vi "RDV-linkPlotVisibility.vi"(8 "error in (no error)":errorcluster, 11 "RDV-Reflection_Data_viewer in":refnum<class "RDV-Reflection_Data_viewer.lvclass">) -> (0 "error out":errorcluster, 3 "RDV-Reflection_Data_viewer out":refnum<class "RDV-Reflection_Data_viewer.lvclass">)   [LabVIEW 2020, in "RDV-Reflection_Data_viewer.lvclass"]
doc: "Links the plot visibility between the viewer's graphs."
uses:
  RDV-Reflection_Data_viewer.lvclass
  RDV-Reflection_Data_viewer.lvclass/RDV-Reflection_Data_viewer.ctl
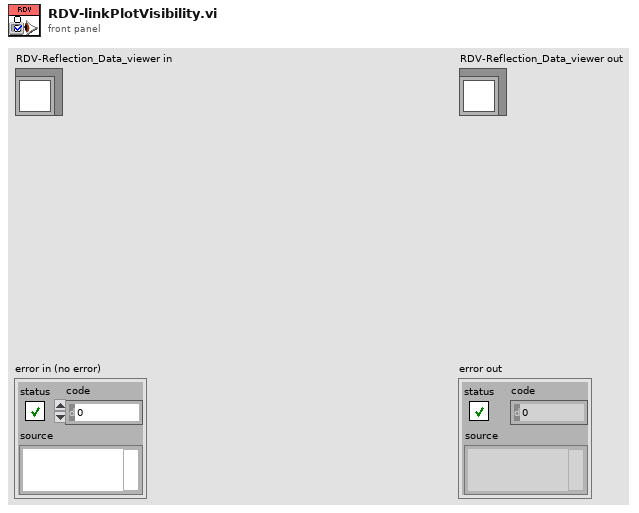
[diagram p1: front panel]
types:
  T1 = typedef "RDV-Reflection_Data_viewer.lvclass/RDV-XY_GRAPH_REFS.ctl" = cluster{"Reflection Real":refnum<vi>, "Reflection Imag":refnum<vi>, "Permittivity Real":refnum<vi>, "Permittivity Imag":refnum<vi>, "Impedance Real":refnum<vi>, "Impedance Imag":refnum<vi>}
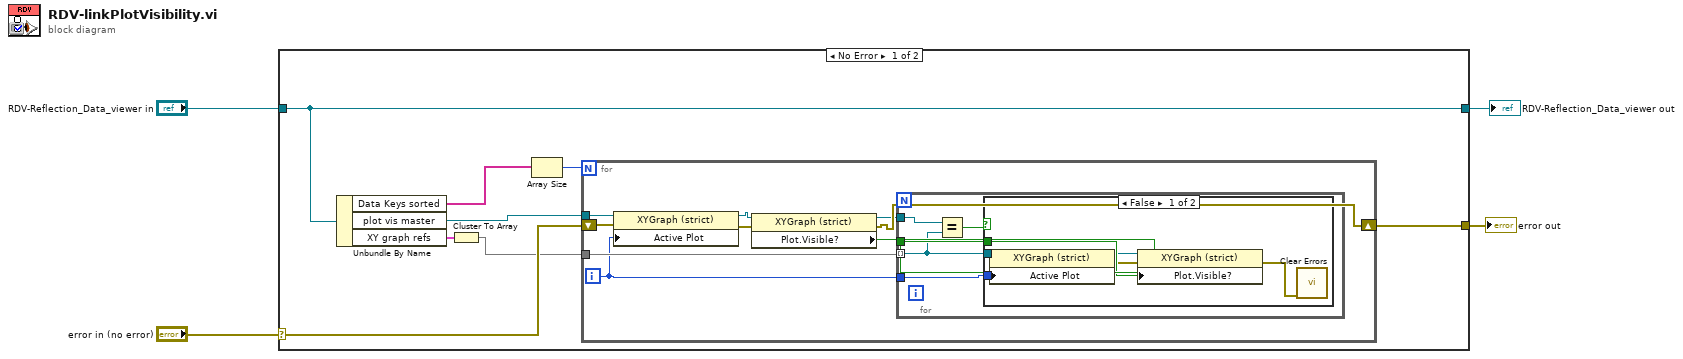
[diagram p0: block diagram]
diagram:
  n1 = case shown="No Error" "error in (no error)" {
    selector: "error in (no error)" -> [w8 w34]
    tunnel: [w9 w34] -> w3
    tunnel: [w12 w33] -> w1
    tunnel: "RDV-Reflection_Data_viewer in" -> [w12 w33]
    frame No Error {
      n2 = Unbundle By Name(w12) -> ("Data Keys sorted"=w11:string[], "plot vis master"=w7:refnum<vi>, "XY graph refs"=w6:T1)
      n3 = Cluster To Array(cluster=w6) -> (array=w5:refnum<vi>[])
      n4 = Array Size(array=w11) -> (size(s)=w10:i32)
      n5 = for {
        N: w10 -> [_]
        tunnel: w5 -> [w21]
        tunnel: w7 -> [w19]
        shift-right: [w14] -> w9
        shift-left: w8 -> [w15]
        i -> [w17]
        n6 = property on="Property Node" class="XYGraph (strict)"(reference=w19, error in=w15, "Active Plot"=w17) -> (reference out=w18:refnum<vi>, error out=w16:errorcluster)
        n7 = property on="Property Node" class="XYGraph (strict)"(reference=w18, error in=w16) -> (reference out=w13:refnum<vi>, error out=w14:errorcluster, "Plot.Visible?"=w20:bool)
        n8 = for {
          tunnel: w20 -> [w26]
          tunnel: w21 -> [w23] mode=indexing
          tunnel: w17 -> [w25]
          tunnel: w13 -> [w24]
          n9 = Equal?(x=w24, y=w23) -> (x = y?=w22:bool)
          n10 = case shown="False" w22 {
            tunnel: w26 -> [w32 _]
            tunnel: w25 -> [w29 _]
            tunnel: w23 -> [w27 _]
            frame False {
              n11 = property on="Property Node" class="XYGraph (strict)"(reference=w27, "Active Plot"=w29) -> (reference out=w31:refnum<vi>, error out=w30:errorcluster)  [unwired: 1 in]
              n12 = property on="Property Node" class="XYGraph (strict)"(reference=w31, error in=w30, "Plot.Visible?"=w32) -> (error out=w28:errorcluster)  [unwired: 1 out]
              n13 = call <vilib>:"Clear Errors.vi"("error in (no error)"=w28) -> ()  [unwired: 5 in, 2 out]
            }
            frame True {
            }
          }
        }
      }
    }
    frame Error {
    }
  }
  "error out" <- w3
  "RDV-Reflection_Data_viewer out" <- w1
